vi "Start Logger.vi"(8 "error in (no error)":errorcluster, 11 "Data Processor Module in":refnum<class "Data Processor Module.lvclass">) -> (0 "error out":errorcluster, 3 "Data Processor Module out":refnum<class "Data Processor Module.lvclass">)   [LabVIEW 2020, in "VolatusData.lvlib" / "Data Processor Module.lvclass"]
uses:
  Data Processor Module.lvclass
  Data Processor Module.lvclass/Data Processor Module.ctl
  Data Logger DBL Module/Data Logger DBL Module.lvclass
  Volatus/Module/Module.lvclass
  VolatusConfig/VolatusConfigElement/VolatusConfigElement.lvclass
  lv-cdm/CDM-Config/Config Element/Config Element.lvclass
  lv-vecto/Vecto/Group/Group.lvclass
  lv-vecto/Vecto/Group DBL/Group DBL.lvclass
  lv-vecto/Vecto/Group BOOL/Group BOOL.lvclass
  C:/dev/lv20CE/relink/lv-volatus/Volatus/Module/Module.lvclass
  Data Logger BOOL Module/Data Logger BOOL Module.lvclass
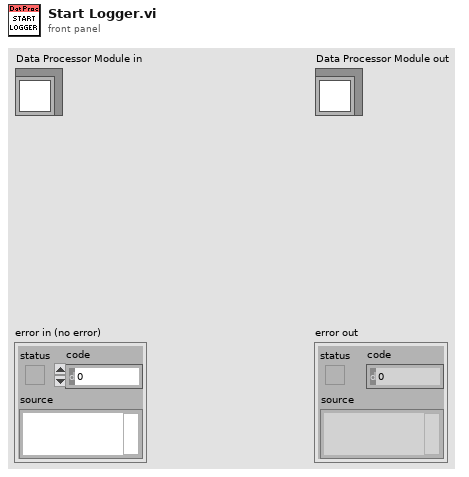
[diagram p1: front panel]
types:
  T1 = typedef "VectoConfig.lvlib/Group Data Type.ctl" = enum16{"Double", "String", "Bool"}
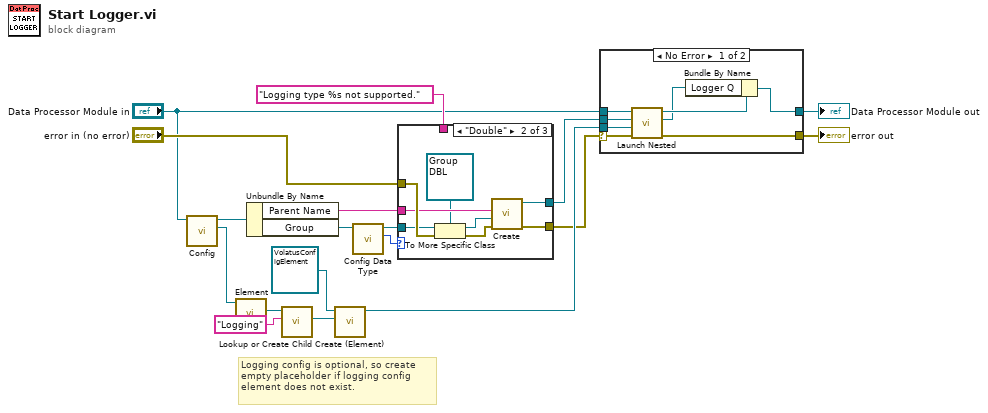
[diagram p0: block diagram]
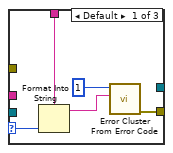
[diagram p2: hidden frame]
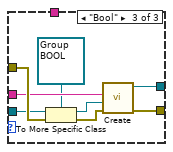
[diagram p3: hidden frame]
diagram:
  # "Logging config is optional, so create empty placeholder if logging config element does not exist."
  n1 = call "Config.vi"("Module in"="Data Processor Module in") -> ("Config"=w13:refnum<class "VolatusConfigElement.lvclass">, "Module out"=w14:refnum<class "Data Processor Module.lvclass">)  [unwired: 9 in]
  n2 = call "Element.vi"("VolatusConfigElement in"=w13) -> ("Element"=w12:refnum<class "Config Element.lvclass">)  [unwired: 9 in, 1 out]
  n3 = Unbundle By Name(w14) -> ("Parent Name"=w17:string, "Group"=w7:refnum<class "Group.lvclass">)
  n4 = call "Lookup or Create Child.vi"("Name"="Logging", "Config Element in"=w12) -> ("Child"=w10:refnum<class "Config Element.lvclass">)  [unwired: 6 in, 3 out]
  n5 = call "Create (Element).vi"("Element"=w10, "VolatusConfigElement in"=refnum<class "VolatusConfigElement.lvclass"> refnum ("Config Element")) -> ("VolatusConfigElement out"=w8:refnum<class "VolatusConfigElement.lvclass">)  [unwired: 8 in, 1 out]
  n6 = call "Config Data Type.vi"("Group in"=w7) -> ("Group Data Type"=w3:T1, "Group out"=w6:refnum<class "Group.lvclass">)  [unwired: 8 in, 1 out]
  n7 = case shown="\"Double\"" w3 {
    selector: w3 -> [w22 _ _]
    tunnel: "error in (no error)" -> [_ w31 w39]
    tunnel: w17 -> [_ w30 w38]
    tunnel: w6 -> [_ w29 w37]
    tunnel: [w23 w28 w36] -> w5
    tunnel: [_ w27 w35] -> w4
    tunnel: "Logging type %s not supported." -> [w21 _ _]
    frame Default {
      n8 = Format Into String(format string=w21, w22) -> (resulting string=w20:string)  [unwired: 2 in, 1 out]
      n9 = call <vilib>:"Error Cluster From Error Code.vi"("error message (\"\")"=w20, "error code (0)"=1) -> ("error out"=w23:errorcluster)  [unwired: 7 in]
    }
    frame "Double" {
      n10 = To More Specific Class(target class=refnum<class "Group DBL.lvclass"> refnum ("Vecto.lvlib:Group DBL.lvclass"), reference=w29, error in=w31) -> (specific class reference=w24:refnum<class "Group DBL.lvclass">, error out=w26:errorcluster)
      n11 = call "Create.vi"("error in (no error)"=w26, "Group"=w24, "Parent Name"=w30) -> ("error out"=w28:errorcluster, "Data Logger Module out"=w27:refnum<class "Data Logger DBL Module.lvclass">)  [unwired: 7 in]
    }
    frame "Bool" {
      n12 = To More Specific Class(target class=refnum<class "Group BOOL.lvclass"> refnum ("Vecto.lvlib:Group BOOL.lvclass"), reference=w37, error in=w39) -> (specific class reference=w32:refnum<class "Group BOOL.lvclass">, error out=w34:errorcluster)
      n13 = call "Create.vi"("error in (no error)"=w34, "Group"=w32, "Parent Name"=w38) -> ("error out"=w36:errorcluster, "Data Logger BOOL Module out"=w35:refnum<class "Data Logger BOOL Module.lvclass">)  [unwired: 7 in]
    }
  }
  n14 = case shown="No Error" w5 {
    selector: w5 -> [w43 w48]
    tunnel: [w47 w48] -> w16
    tunnel: [w46 w49] -> w15
    tunnel: "Data Processor Module in" -> [w45 w49]
    tunnel: w8 -> [w44 _]
    tunnel: w4 -> [w41 _]
    frame No Error {
      n15 = call "Launch Nested.vi"("error in (no error)"=w43, "Config Element"=w44, "Nested Module"=w41, "Parent in"=w45) -> ("error out"=w47:errorcluster, "MessageQ"=w40:refnum<class "MessageQ.lvclass">, "Parent out"=w42:refnum<class "Data Processor Module.lvclass">)  [unwired: 5 in]
      n16 = Bundle By Name(cluster=w42, "Logger Q"=w40) -> (w46:refnum<class "Data Processor Module.lvclass">)
    }
    frame Error {
    }
  }
  "error out" <- w16
  "Data Processor Module out" <- w15
